vi "Element Events.vi"(8 "error in (no error)":errorcluster, 11 "NumericCommandButton in":refnum<class "NumericCommandButton.lvclass">) -> (0 "error out":errorcluster, 2 "Element Events":refnum<class "Control Event Registrations.lvclass">, 3 "NumericCommandButton out":refnum<class "NumericCommandButton.lvclass">)   [LabVIEW 2025, in "VolatusGUIElements.lvlib" / "NumericCommandButton.lvclass"]
uses:
  NumericCommandButton.lvclass
  VolatusGUI/Control Event Registrations/Control Event Registrations.lvclass
  NumericCommandButton.lvclass/NumericCommandButton.ctl
  C:/dev/volatus/mts-volatus-super/libs/lv-volatus/VolatusGUI/GUI Element/GUI Element.lvclass
  C:/dev/volatus/mts-volatus-super/libs/lv-volatus/VolatusGUIElements/NumericCommandButton/NumericCommandButton.lvclass
  C:/dev/volatus/mts-volatus-super/libs/lv-volatus/VolatusGUI/OnValueChangeHandler/OnValueChangeHandler.lvclass
  VolatusGUI/GUI Element/GUI Element.lvclass
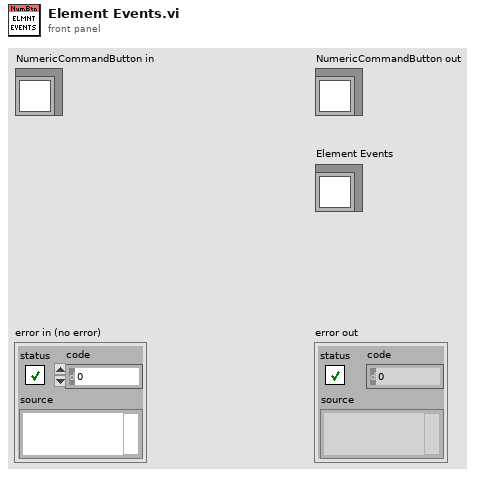
[diagram p1: front panel]
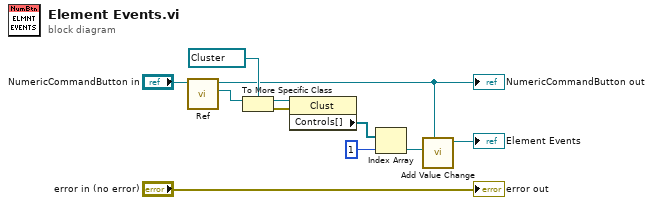
[diagram p0: block diagram]
diagram:
  n1 = call "Ref.vi"("GUI Element in"="NumericCommandButton in") -> ("Ref"=w7:refnum<vi>, "GUI Element out"=w3:refnum<class "NumericCommandButton.lvclass">)  [unwired: 9 in]
  "NumericCommandButton out" <- w3
  n2 = To More Specific Class(target class=refnum<vi> refnum ("specific class reference"), reference=w7) -> (specific class reference=w9:refnum<vi>, error out=w8:errorcluster)  [unwired: 1 in]
  n3 = property class="Clust"(reference=w9, error in=w8) -> ("Controls[]"=w6:refnum<vi>[])  [unwired: 2 out]
  n4 = Index Array(array=w6, index=1) -> (element=w2:refnum<vi>)
  n5 = call "Add Value Change.vi"("Control"=w3, "CtlRef"=w2) -> ("Control Event Registrations out"=→"Element Events":refnum<class "Control Event Registrations.lvclass">)  [unwired: 8 in, 1 out]
  "error out" <- "error in (no error)"
